vi "CreateAIO_DAQ_CFG.vi"(8 "error in (no error)":errorcluster, 9 "Data":T1, 10 "Name":string, 11 "object in":refnum<class "AIO-Configuration.lvclass">) -> (0 "error out":errorcluster, 3 "object out":refnum<class "AIO-Configuration.lvclass">)   [LabVIEW 2021, in "DAQmx.lvlib" / "AIO-Configuration.lvclass"]
uses:
  AIO-Configuration.lvclass
  C:/Users/averna/Documents/LV Gym DEMO/Factory Pattern/Generic Channel/Configuration/Configuration.lvclass
  tdef/Data.ctl
  AIO-Configuration.lvclass/AIO-Configuration.ctl
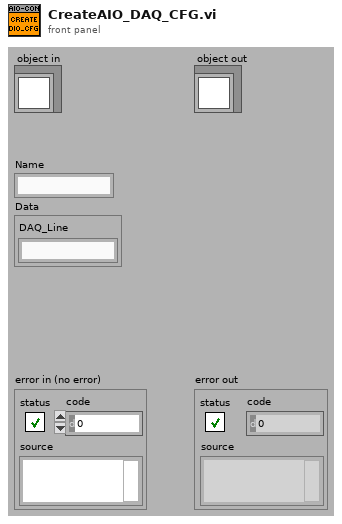
[diagram p1: front panel]
types:
  T1 = typedef "DAQmx.lvlib/AIO-Configuration.lvclass/Data.ctl" = cluster{"DAQ_Line":string}
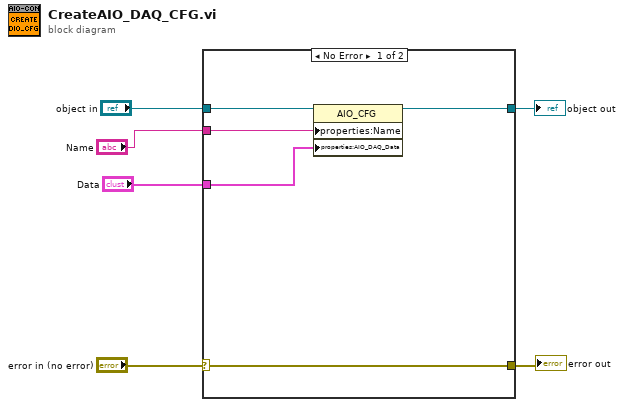
[diagram p0: block diagram]
diagram:
  n1 = case shown="No Error" "error in (no error)" {
    selector: "error in (no error)" -> [w11 w13]
    tunnel: [w11 w13] -> w5
    tunnel: [w9 w12] -> w3
    tunnel: "object in" -> [w10 w12]
    tunnel: "Name" -> [w8 _]
    tunnel: "Data" -> [w7 _]
    frame No Error {
      n2 = property class="AIO_CFG"(reference=w10, "properties:Name"=w8, "properties:AIO_DAQ_Data"=w7) -> (reference out=w9:refnum<class "AIO-Configuration.lvclass">)  [unwired: 1 in, 1 out]
    }
    frame Error {
    }
  }
  "error out" <- w5
  "object out" <- w3
